vi "RemoteVI Wait Highlight Change.vi"(0 "menu":u64, 5 "found before":bool, 7 "top before":i32=-1, 9 "timeout ms":u32=120, 11 "error in":errorcluster) -> (4 "changed?":bool, 15 "error out":errorcluster)   [LabVIEW 2020, in "RemoteVI.lvlib"]
doc: "After a key was posted to an open LabVIEW menu, waits until the menu shows the result: captures the menu window (RemoteVI Menu Highlight.vi) every 5 ms until its highlight differs from the one before the key (found before, top before) or timeout ms have passed. LabVIEW has handled the key when the WM_NULL round trip returns, but its repaint of the menu can come later: captured right away from the server loop, the old highlight was seen for over 100 ms (measured), so reading it once made the navigation stop one item short. Returns at once when the highlight already changed. changed? is FALSE after a timeout - the key moved nothing (an end of the menu, or a window that takes no keys). Win32 only, no VI Server call."
uses:
  RemoteVI.lvlib
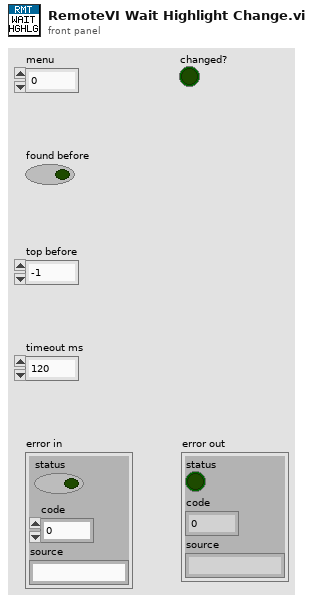
[diagram p1: front panel]
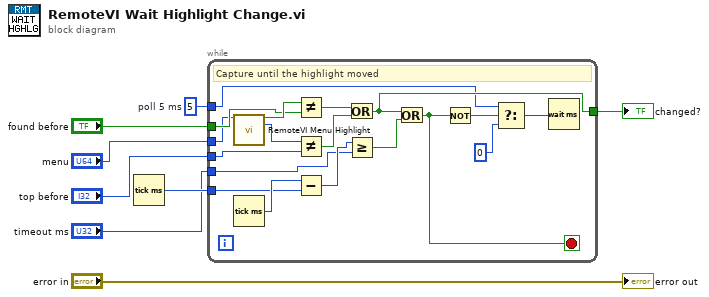
[diagram p0: block diagram]
diagram:
  w7 = u32 5  # poll 5 ms
  n1 = Tick Count (ms)() -> (millisecond timer value=w6:u32)
  n2 = while {
    tunnel: "menu" -> [w9]
    tunnel: "found before" -> [w10]
    tunnel: "top before" -> [w11]
    tunnel: "timeout ms" -> [w12]
    tunnel: w7 -> [w14]
    tunnel: w6 -> [w13]
    tunnel: [w19] -> w8
    stop <- w23 stop-if-true
    # "Capture until the highlight moved"
    n3 = call "RemoteVI Menu Highlight.vi"("hwnd"=w9) -> ("found?"=w15:bool, "top"=w16:i32)  [unwired: 9 in, 4 out]
    n4 = Tick Count (ms)() -> (millisecond timer value=w20:u32)
    n5 = Not Equal?(x=w15, y=w10) -> (x != y?=w17:bool)
    n6 = Not Equal?(x=w16, y=w11) -> (x != y?=w18:bool)
    n7 = Subtract(x=w20, y=w13) -> (x-y=w21:u32)
    n8 = Or(x=w17, y=w18) -> (x .or. y?=w19:bool)
    n9 = Greater Or Equal?(x=w21, y=w12) -> (x >= y?=w22:bool)
    n10 = Or(x=w19, y=w22) -> (x .or. y?=w23:bool)
    n11 = Not(x=w23) -> (.not. x?=w24:bool)
    n12 = Select(t=w14, s=w24, f=u32 0) -> (s? t:f=w26:u32)
    n13 = Wait (ms)(milliseconds to wait=w26) -> ()  [unwired: 1 out]
  }
  "changed?" <- w8
  "error out" <- "error in"
